vi "Read outputFolder.vi"(8 "error in (no error)":errorcluster, 11 "ZM-CP-FL-file_logger in":refnum<class "ZM-CP-FL-file_logger.lvclass">) -> (0 "error out":errorcluster, 2 "outputFolder":path, 3 "ZM-CP-FL-file_logger out":refnum<class "ZM-CP-FL-file_logger.lvclass">)   [LabVIEW 2020, in "ZM-CP-FL-file_logger.lvlib" / "ZM-CP-FL-file_logger.lvclass"]
doc: "Reads one field of this class's private data. Generated by lvai_create_accessors from the class private data control."
uses:
  ZM-CP-FL-file_logger.lvclass
  ZM-CP-FL-file_logger.lvclass/ZM-CP-FL-file_logger.ctl
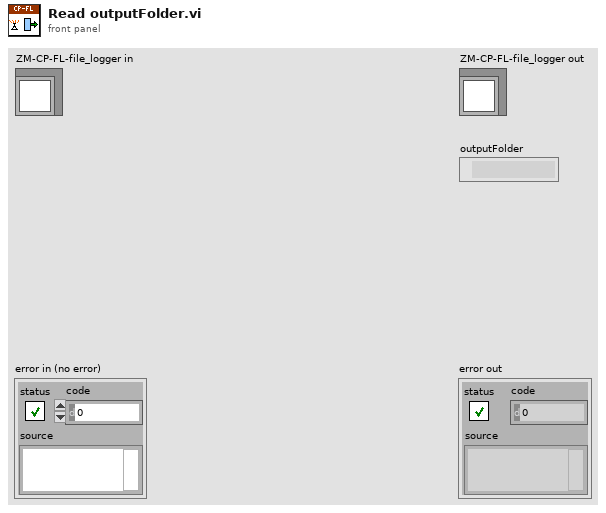
[diagram p1: front panel]
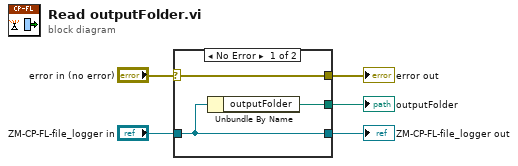
[diagram p0: block diagram]
diagram:
  n1 = case shown="No Error" "error in (no error)" {
    selector: "error in (no error)" -> [w8 w9]
    tunnel: [w8 w9] -> w4
    tunnel: [w7 w10] -> w2
    tunnel: "ZM-CP-FL-file_logger in" -> [w7 w10]
    tunnel: [w6 _] -> w1
    frame No Error {
      n2 = Unbundle By Name(w7) -> ("outputFolder"=w6:path)
    }
    frame Error {
    }
  }
  "error out" <- w4
  "ZM-CP-FL-file_logger out" <- w2
  "outputFolder" <- w1
